vi "Test_case.vi"(7 "base path":path=path "D:/1.INPROGRESS/16.Ather/6.Software/Ather_ANC_LEV_Labview_Software/Template", 9 "Main Test Status":refnum<vi>, 10 "queue out":refnum<queue>, 11 "Data Cluster":T2={"Boolean <Replace Me>"=FALSE, "String <Replace Me>"="", "Numeric <Replace Me>"=0.0, "Do Something Ref"=refnum, "Do Something Else Ref"=refnum, "Data Display Ref"=refnum, "Exit Button Ref"=refnum, "Enum"=enum."Admin", "skip Test  "=[]}) -> (3 "Result":string[][](array[string]))   [LabVIEW 2021]
uses:
  controls/UI Data.ctl
  Main_VI/Control/login_type.ctl
  controls/Main test sequence.ctl
  5.ACTIVITIES/1.LabVIEW_State_Machine_Template/LabVIEW_State_Machine_Template/LabVIEW_State_Machine_Template/Project_Template/Queue Test updator/Controls/initialise cluster.ctl
  5.ACTIVITIES/1.LabVIEW_State_Machine_Template/LabVIEW_State_Machine_Template/LabVIEW_State_Machine_Template/Project_Template/Queue Test updator/Controls/test step description.ctl
  5.ACTIVITIES/1.LabVIEW_State_Machine_Template/LabVIEW_State_Machine_Template/LabVIEW_State_Machine_Template/Project_Template/Queue Test updator/Controls/comparison selection.ctl
panel:
  out "Main test sequence 2":T1
  out "Main test sequence":T1
  out "s? t:f":T1
  out "Test Status 2":i32(listbox)=-1
  out "UI":string[][](array[string])=[["1", "start BB4 card auto testing", "0.000", "0.000", "", ""], ["2", "scan barcode", "0.000", "0.000", "", ""], ["3", "ensure resistor settings", "0.000", "0.000", "", ""], ["4", "check shorting of TP01 wrt GND", "100000.000", "200000.000", "", ""], ["5", "check shorting of TP02 wrt GND", "100000.000", "200000.000", "", ""], ["6", "check shorting of TP05 wrt GND", "100000.000", "200000.000", "", ""], ["7", "check shorting of TP36 wrt GND", "180.000", "200.000", "", ""], ["8", "check shorting of TP42 wrt GND", "240.000", "270.000", "", ""], ["9", "check shorting of TP41 wrt GND", "210.000", "230.000", "", ""], ["10", "check shorting of TP30 wrt GND", "145.000", "155.000", "", ""], ["11", "turn ON 5V PS", "0.000", "0.000", "", ""], ["12", "measure voltage at TP01", "3.200", "3.400", "", ""], ["13", "measure voltage at TP02", "3.200", "3.400", "", ""], ["14", "measure voltage at TP05", "1.600", "1.800", "", ""], ["15", "measure 0.02A current at PS_I/P", "0.010", "0.030", "", ""], ["16", "program UCD9081(JF1)", "0.100", "0.300", "", ""], ["17", "program UCD9081(JF2)", "0.000", "0.000", "", ""], ["18", "program UCD9081(JF3)", "0.000", "0.000", "", ""], ["19", "measure 0.4A current at PS_I/P", "0.350", "0.450", "", ""], ["20", "turn OFF 5V PS", "0.000", "0.000", "", ""], ["21", "measure resistance at C56_C59", "100000.000", "200000.000", "", ""], ["22", "turn ON 5V PS", "0.000", "0.000", "", ""], ["23", "measure voltage at TP36", "1.700", "1.900", "", ""], ["24", "measure voltage at TP42", "3.200", "3.400", "", ""], ["25", "measure voltage at TP41", "1.100", "1.300", "", ""], ["26", "measure voltage at TP30", "2.400", "2.600", "", ""], ["27", "boundary scan test", "0.000", "0.000", "", ""], ["28", "monitor clock I/P of U49.3", "26.500", "27.500", "", ""], ["29", "flash Cypress_CY223811FXI", "0.000", "0.000", "", ""], ["30", "monitor clock I/P of U48.1", "24.500", "25.500", "", ""], ["31", "monitor clock I/P of U48.5", "26.500", "27.500", "", ""], ["32", "monitor clock I/P of U32.2", "24.500", "25.500", "", ""], ["33", "monitor clock I/P of U32.3", "24.500", "25.500", "", ""], ["34", "monitor clock I/P of U32.4", "24.500", "25.500", "", ""], ["35", "monitor clock I/P of U32.5", "24.500", "25.500", "", ""], ["36", "monitor clock I/P of U53.2", "24.500", "25.500", "", ""], ["37", "monitor clock I/P of U53.3", "24.500", "25.500", "", ""], ["38", "monitor clock I/P of U53.4", "24.500", "25.500", "", ""], ["39", "monitor clock I/P of U53.5", "24.500", "25.500", "", ""], ["40", "monitor clock I/P of U233.2", "24.500", "25.500", "", ""], ["41", "monitor clock I/P of U233.3", "24.500", "25.500", "", ""], ["42", "monitor clock I/P of U233.4", "24.500", "25.400", "", ""], ["43", "monitor clock I/P of U233.5", "24.500", "25.500", "", ""], ["44", "monitor clock I/P of U33.2", "26.500", "27.500", "", ""], ["45", "monitor clock I/P of U33.3", "26.500", "27.500", "", ""], ["46", "monitor clock I/P of U33.4", "26.500", "27.500", "", ""], ["47", "monitor clock I/P of U33.5", "26.500", "27.500", "", ""], ["48", "monitor clock I/P of U38.2", "26.500", "27.500", "", ""], ["49", "monitor clock I/P of U38.3", "26.500", "27.500", "", ""], ["50", "monitor clock I/P of U38.4", "26.500", "27.500", "", ""], ["51", "monitor clock I/P of U38.5", "26.500", "27.500", "", ""], ["52", "monitor clock I/P of U46.2", "26.500", "27.500", "", ""], ["53", "monitor clock I/P of U46.3", "26.500", "27.500", "", ""], ["54", "monitor clock I/P of U46.4", "26.500", "27.500", "", ""], ["55", "monitor clock I/P of U46.5", "26.500", "27.500", "", ""], ["56", "monitor reset O/P of U60.1 as 5.0V", "4.800", "5.200", "", ""], ["57", "monitor reset O/P of U36.4 as 5.0V", "4.800", "5.200", "", ""], ["58", "monitor reset O/P of U36.6 as 5.0V", "4.800", "5.200", "", ""], ["59", "monitor reset O/P of U36.8 as 5.0V", "4.800", "5.200", "", ""], ["60", "monitor reset O/P of U36.10 as 5.0V", "4.800", "5.200", "", ""], ["61", "monitor reset O/P of U36.12 as 5.0V", "4.800", "5.200", "", ""], ["62", "user prompt for pressing reset switch SW3 at U60.1", "0.000", "0.000", "", ""], ["63", "user prompt for pressing reset switch SW3 at U36.4", "0.000", "0.000", "", ""], ["64", "user prompt for pressing reset switch SW3 at U36.6", "0.000", "0.000", "", ""], ["65", "user prompt for pressing reset switch SW3 at U36.8", "0.000", "0.000", "", ""], ["66", "user prompt for pressing reset switch SW3 at U36.10", "0.000", "0.000", "", ""], ["67", "user prompt for pressing reset switch SW3 at U36.12", "0.000", "0.000", "", ""], ["68", "program FPGA via .bit file", "0.000", "0.000", "", ""], ["69", "FPGA SPI flash via .mcs file", "0.000", "0.000", "", ""], ["70", "Ethernet test_Portxx", "0.000", "0.000", "", ""], ["71", "JTAG connectivity of DAVINCI (SMS320DM6446AZWTA)", "0.000", "0.000", "", ""], ["72", "UBOOT test_DVflasher", "0.000", "0.000", "", ""], ["73", "UBOOT test_send command on hyperterminal and verify result", "0.000", "0.000", "", ""], ["74", "Send Kernel_INDESDR", "0.000", "0.000", "", ""], ["75", "Send NAND Erase_Write_Boot", "0.000", "0.000", "", ""], ["76", "Send_nci_nce_ncn", "0.000", "0.000", "", ""], ["77", "Muti IDE", "0.000", "0.000", "", ""], ["78", "FileZilla File System Transfer", "0.000", "0.000", "", ""], ["79", "Telnet Unmount Device", "0.000", "0.000", "", ""], ["80", "Ethernet test_Portxx", "0.000", "0.000", "", ""], ["81", "LAN9250 test", "0.000", "0.000", "", ""], ["82", "ping IP_LAN9250 test", "0.000", "0.000", "", ""], ["83", "RTC Test", "0.000", "0.000", "", ""], ["84", "Shared Memory Test", "0.000", "0.000", "", ""], ["85", "Temperature_Sensor_Test", "0.000", "0.000", "", ""], ["86", "GPS_Test", "0.000", "0.000", "", ""], ["87", "External Clock Test", "0.000", "0.000", "", ""], ["88", "stop BB4 card auto testing", "0.000", "0.000", "", ""]]
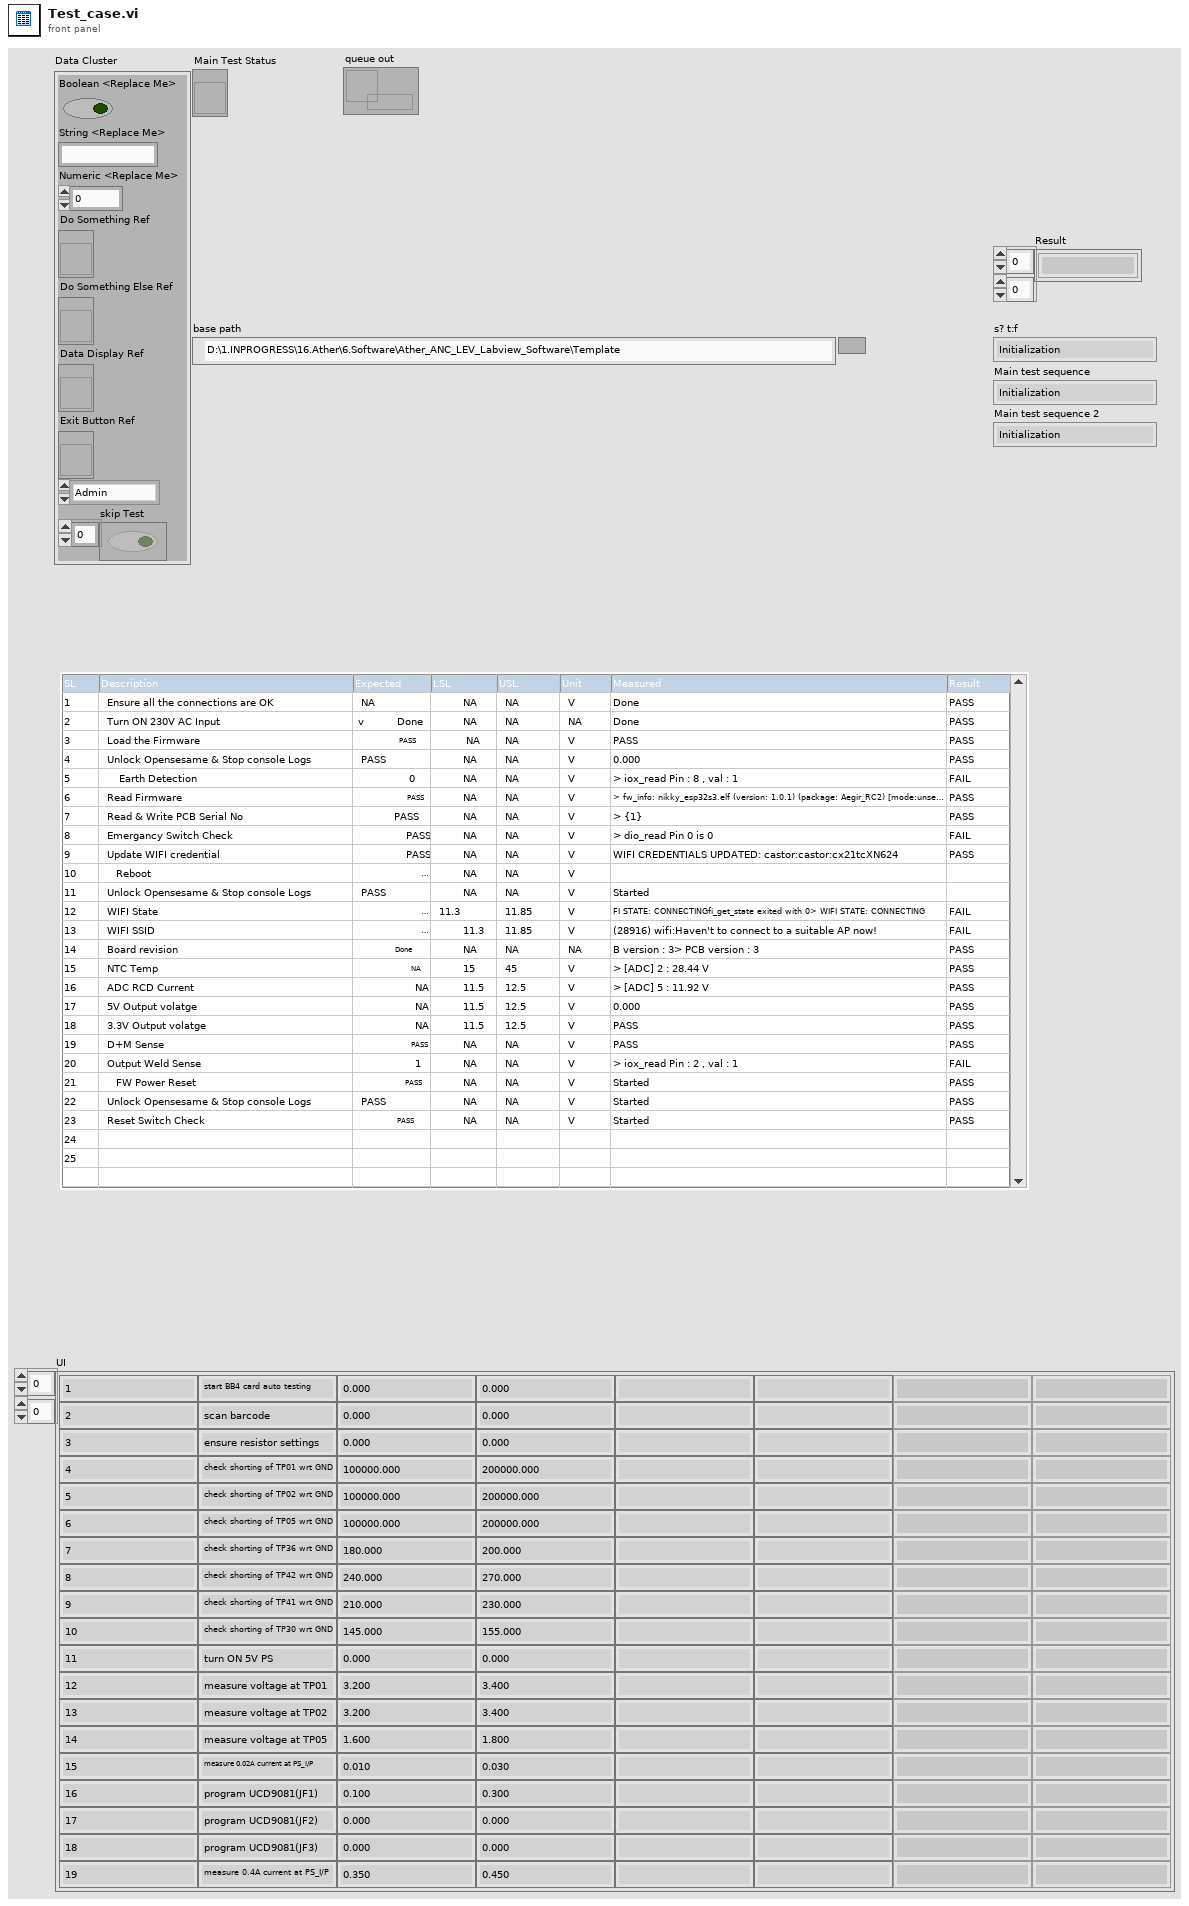
[diagram p1: front panel]
types:
  T1 = typedef "Main test sequence.ctl" = enum16{"Initialization", "Ensure all the connections are OK", "Turn ON 230V AC Input", "Load the Firmware", "Unlock_Opensesame & Stop console Logs", "Earth Detection", "Read Firmware", "Read & Write PCB Serial No", "Emergancy Switch Check", "Update WIFI credentials ", "Reboot", "Unlock Opensesame & Stop_console Logs", "WIFI State", "WIFI SSID", "Board revision", "ADC NTC Temp", "ADC_TYPE2_RCD_CURRENT", "5V Output Voltage", "3.3V Output Voltage", "D+M Sense", "Output Weld Sense", "FW Power Reset", "Unlock Opensesame & Stop console_Logs", "Reset switch Check", "Exit"}
  T2 = typedef "UI Data.ctl" = cluster{"Boolean <Replace Me>":bool, "String <Replace Me>":string, "Numeric <Replace Me>":dbl, "Do Something Ref":refnum<vi>, "Do Something Else Ref":refnum<vi>, "Data Display Ref":refnum<vi>, "Exit Button Ref":refnum<vi>, "Enum":T3, "skip Test  ":bool[]}
  T3 = typedef "login_type.ctl" = enum16{"Operator", "Admin"}
  T4 = typedef "initialise cluster.ctl" = cluster{"User name":string, "user account":string, "UI":string[][], "DI":T5[], "Barcode":string, "MCListbox Ref_in":refnum<vi>, "sequence step #":u32, "Result?":bool, "Report Path":path, "Test Sequence":T1, "skip Test  ":bool[]}
  T5 = typedef "test step description.ctl" = cluster{"Lower limit":dbl, "Upper limit":dbl, "Comparison":T6, "Expected":string, "Enable":bool, "Main test sequence":T1}
  T6 = typedef "comparison selection.ctl" = enum16{"None", "in-range?", "less than?", "greater than?", "equal to?", "not equal to?", "less or equal to?", "greater or equal to?"}
  T7 = typedef "initialise cluster.ctl" = cluster{"User name":string, "user account":string, "UI":string[][], "DI":T8[], "Skip test?":bool[], "Barcode":string, "MCListbox Ref_in":refnum<vi>, "sequence step #":u32, "Result?":bool, "Report Path":path, "Enum":T10}
  T8 = typedef "test step description.ctl" = cluster{"Test_Sequence":T9, "Lower limit":dbl, "Upper limit":dbl, "Comparison":T6, "Expected":string, "Enable":bool}
  T9 = typedef "Test_sequence.ctl" = enum16{"Init Devices", "Login", "Option Window", "Idle state", "Scan Barcode", "Clear the test Containers", "Init-Pre Test", "Test ", "Result", "Report", "Database", "Update Display", "Confirm Quit", "Error", "Exit"}
  T10 = typedef "Test_Sequence_4.ctl" = enum16{"Update Display", "User Login", "Operator", "Admin", "Developer", "Update Test Seq", "Initialise", "Init Devices", "Idle State", "Check All", "UnCheck All", "Abort", "Start Testing", "Turn ON Power", "Scan Barcode", "POP to place DUT", "Toggle Operation confirmation", "Error", "Confirm Quit", "Exit", "Code flash", "Operating Voltage range test", "Under Voltage Protection", "Reverse Voltage Test at 28V", "Reverse Voltage Recovery", "Output Test at 8V", "Output Test at 9V", "Output Test at 10V", "Output Test at 11V", "Output Test at 12V", "Output Test at 15V", "Output Test at 24V", "Output Test at 32V", "Video Signal Conversion Test", "USB Interface Verification", "Turn OFF Power", "Report"}
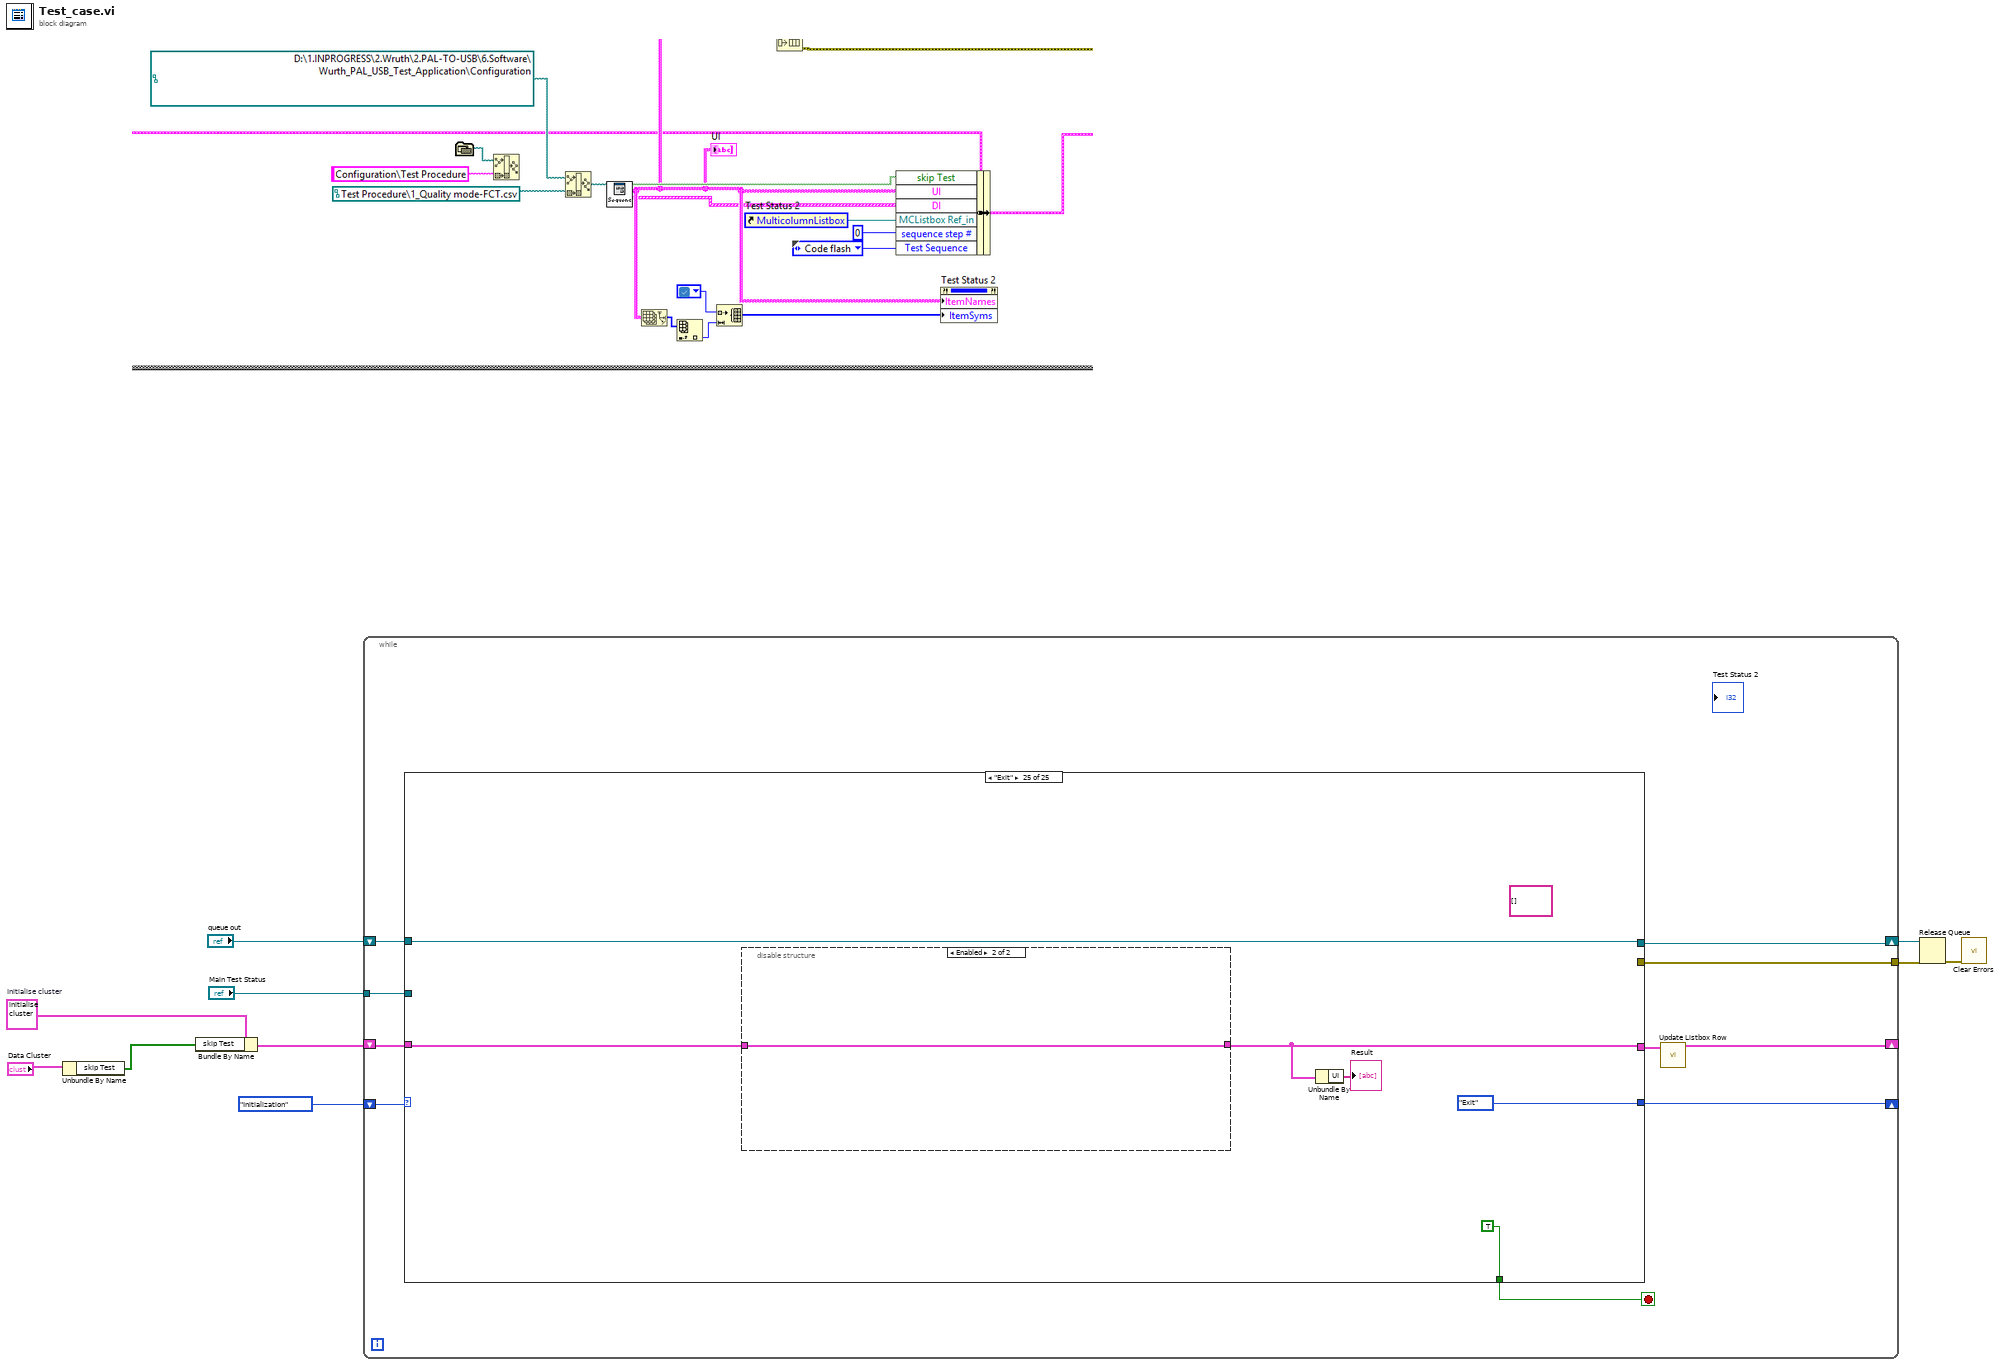
[diagram p0: block diagram]
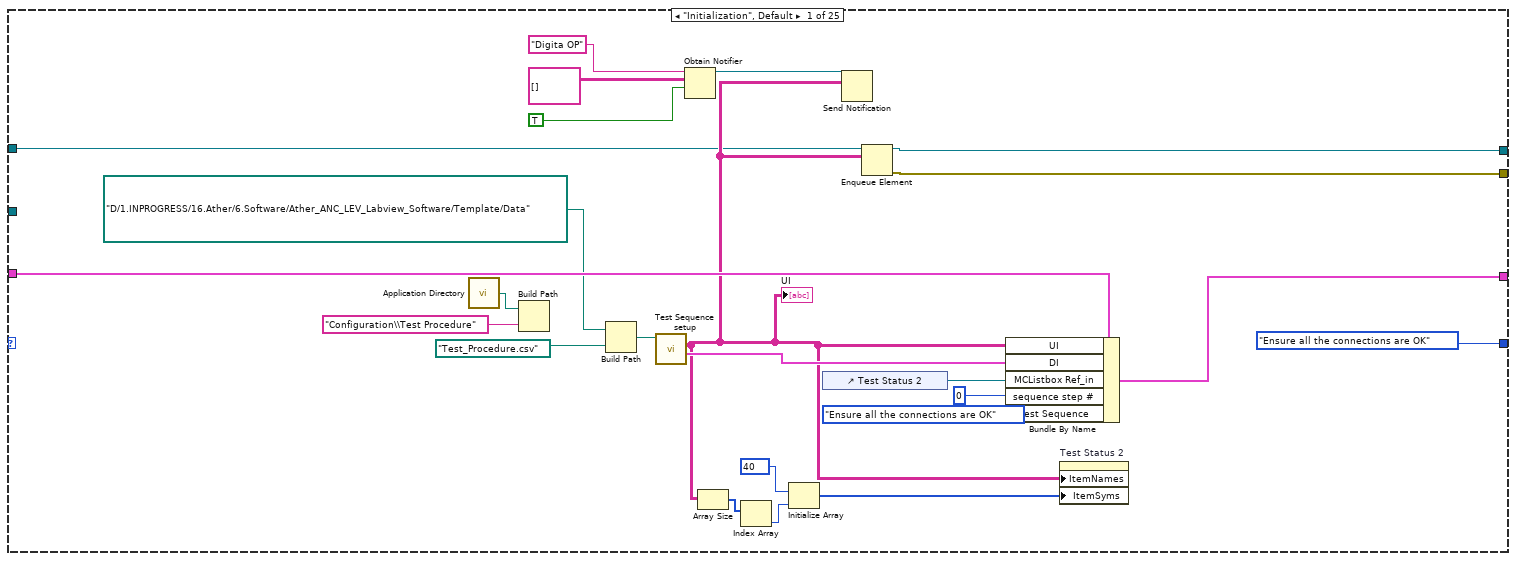
[diagram p2: hidden frame]
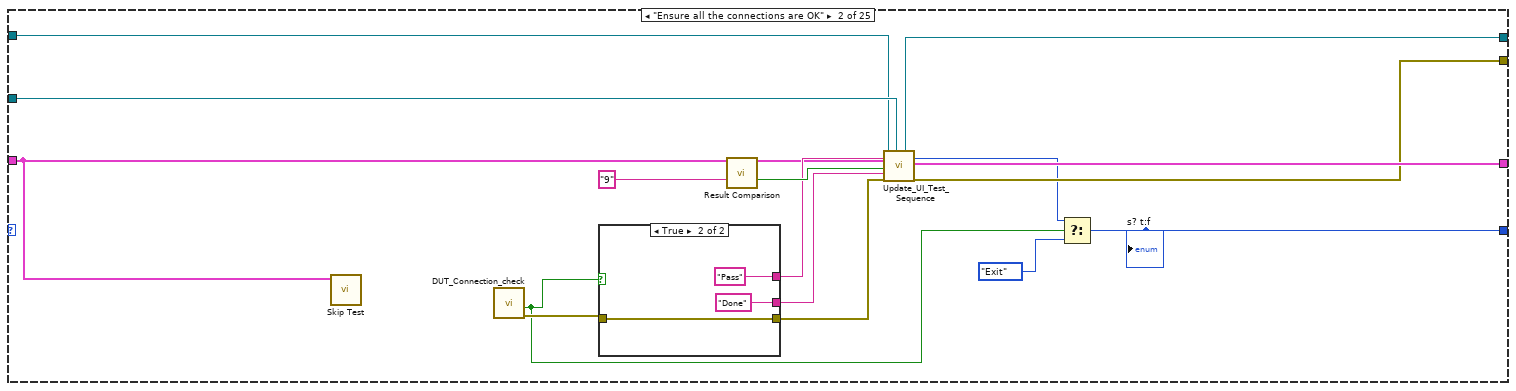
[diagram p3: hidden frame]
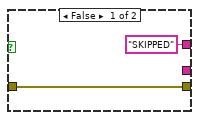
[diagram p4: hidden frame]
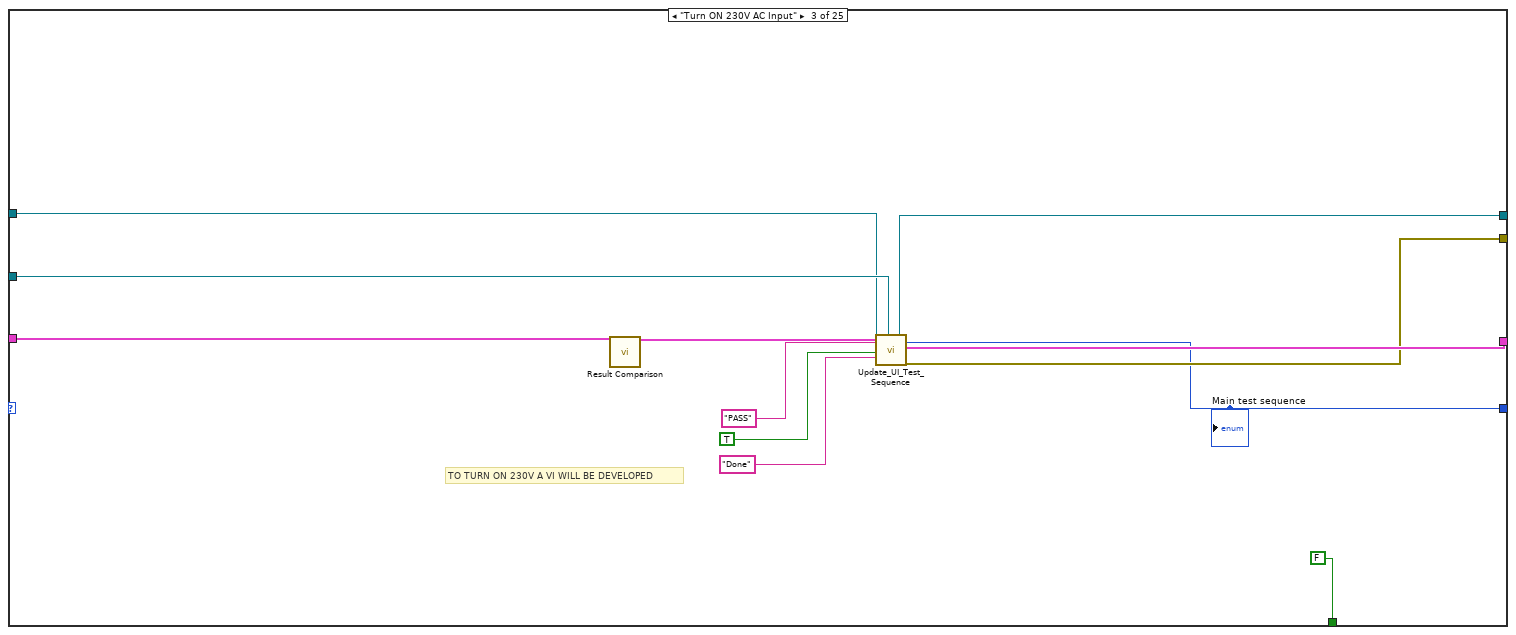
[diagram p5: hidden frame]
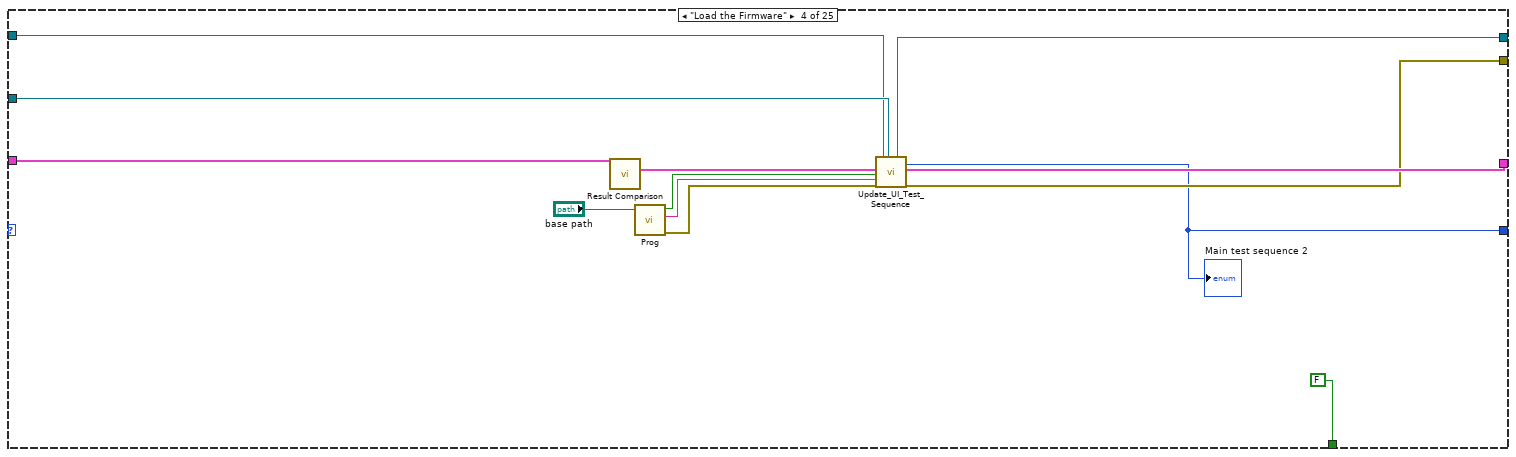
[diagram p6: hidden frame]
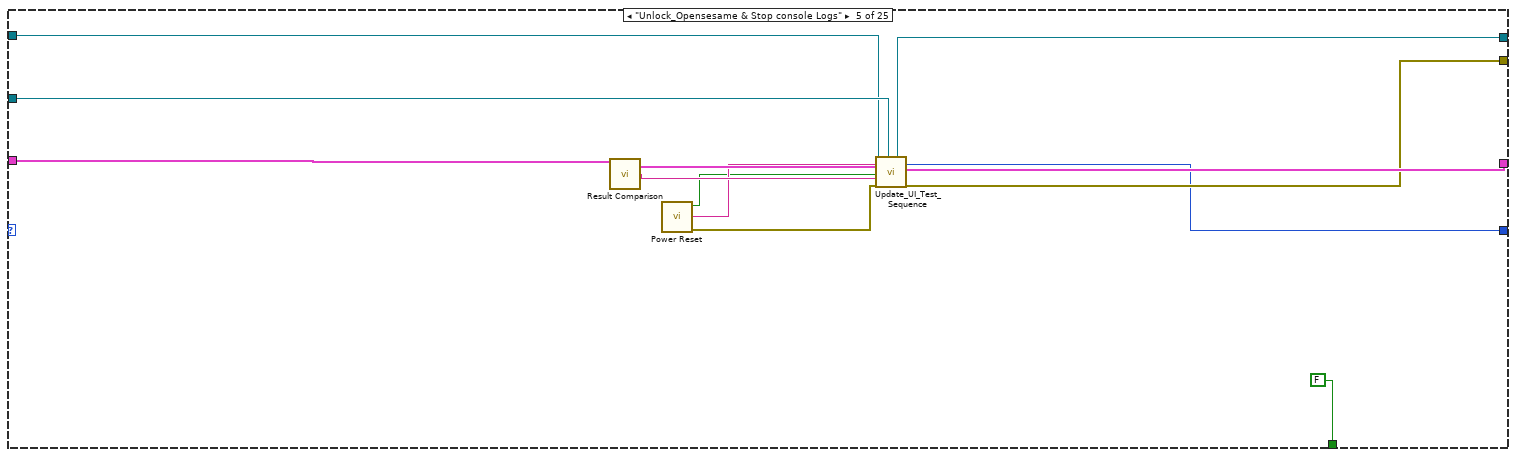
[diagram p7: hidden frame]
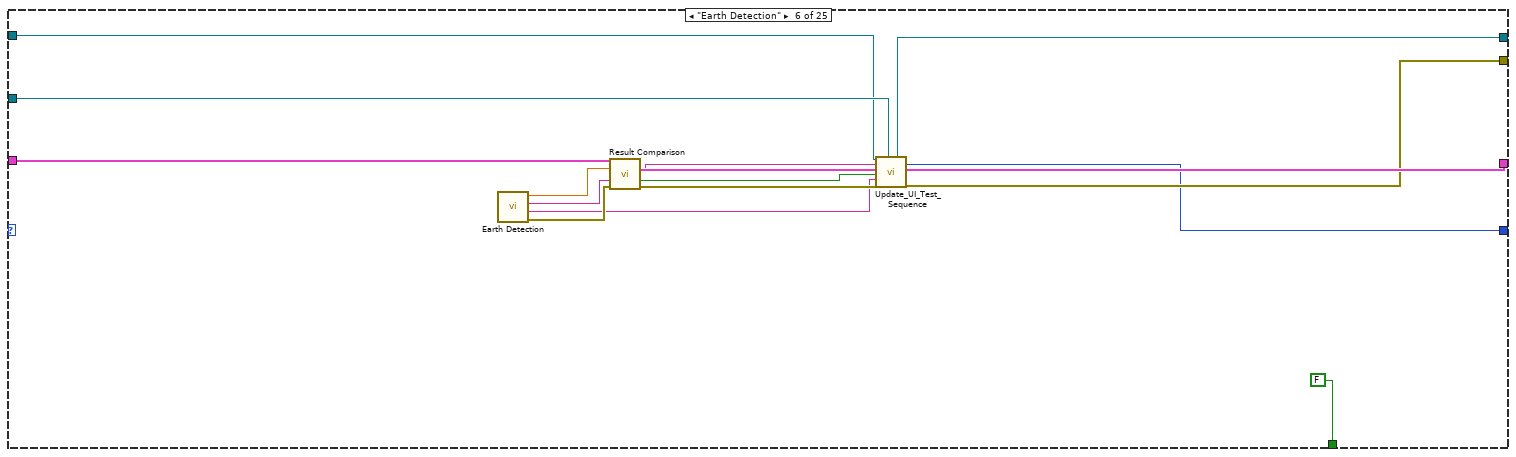
[diagram p8: hidden frame]
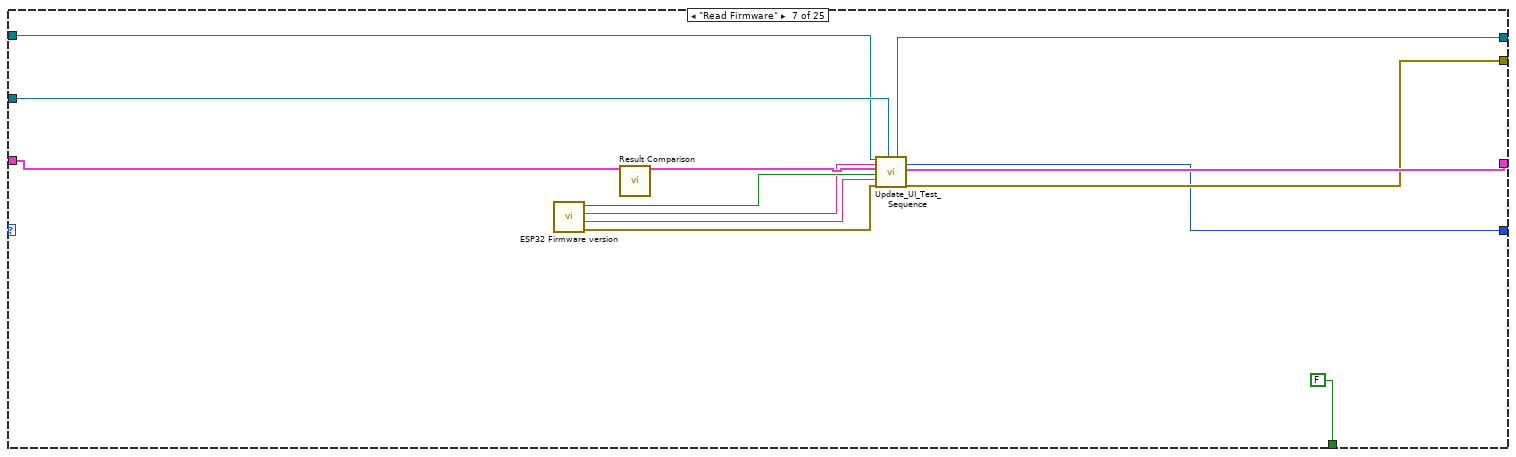
[diagram p9: hidden frame]
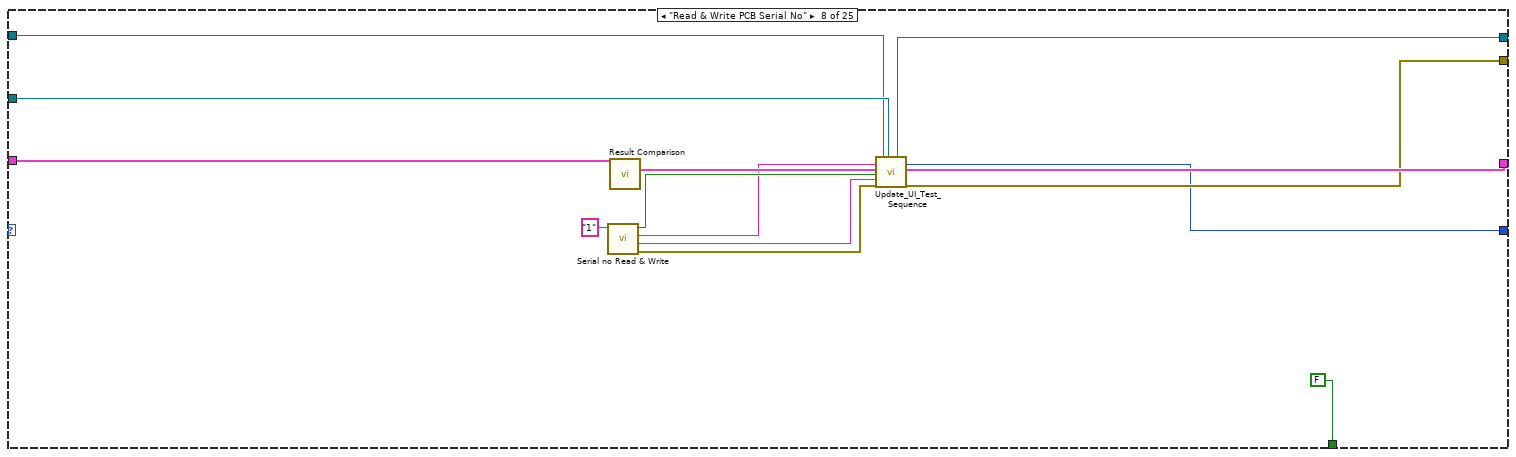
[diagram p10: hidden frame]
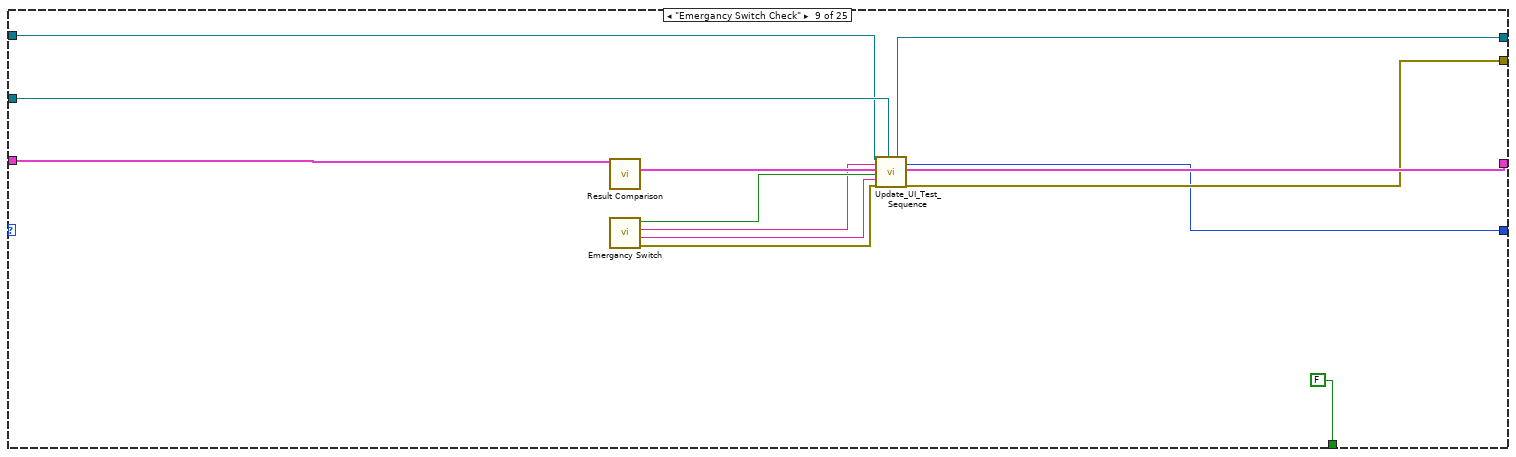
[diagram p11: hidden frame]
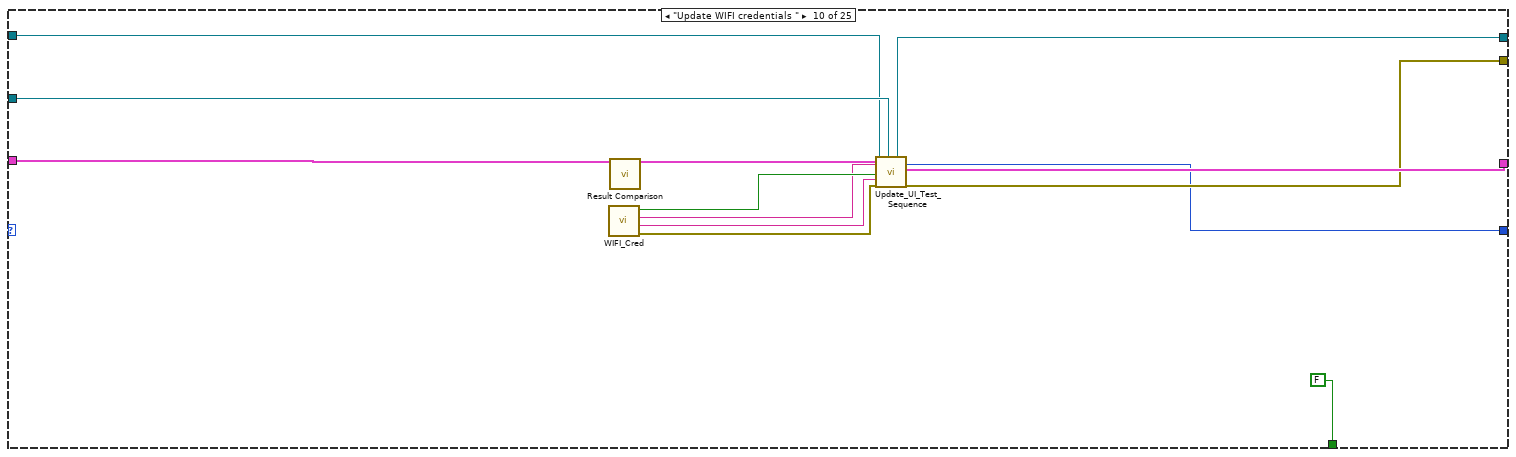
[diagram p12: hidden frame]
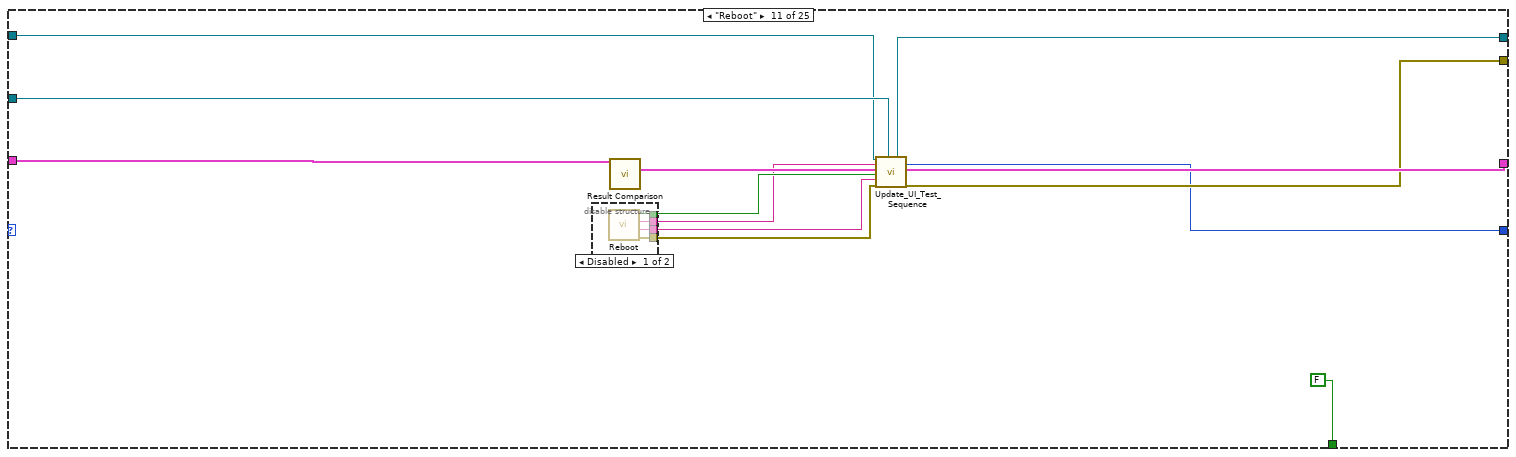
[diagram p13: hidden frame]
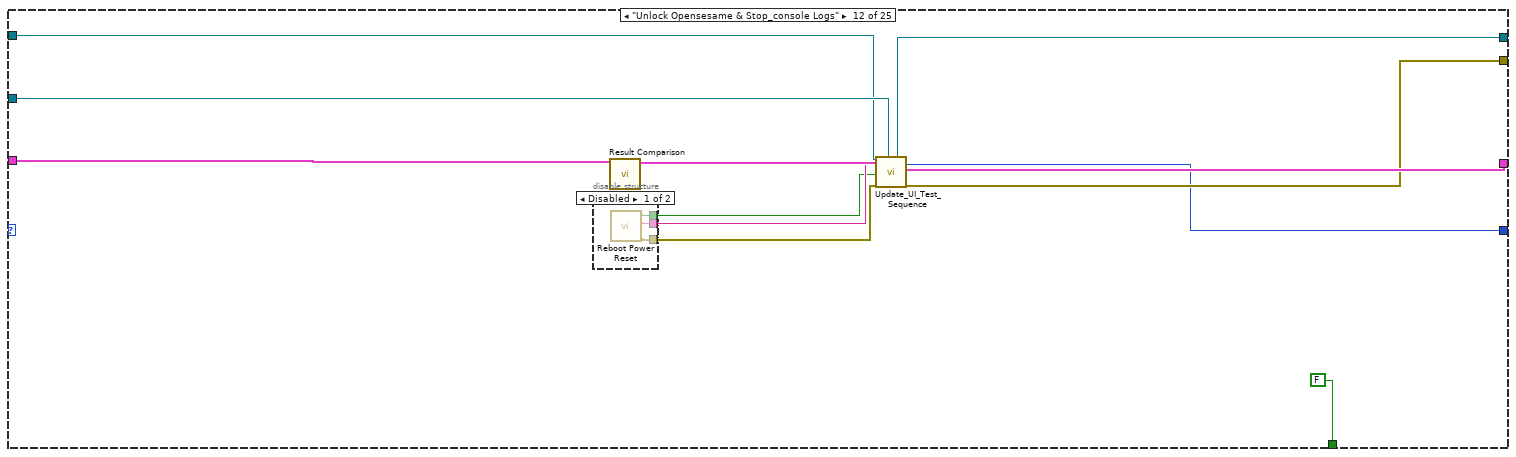
[diagram p15: hidden frame]
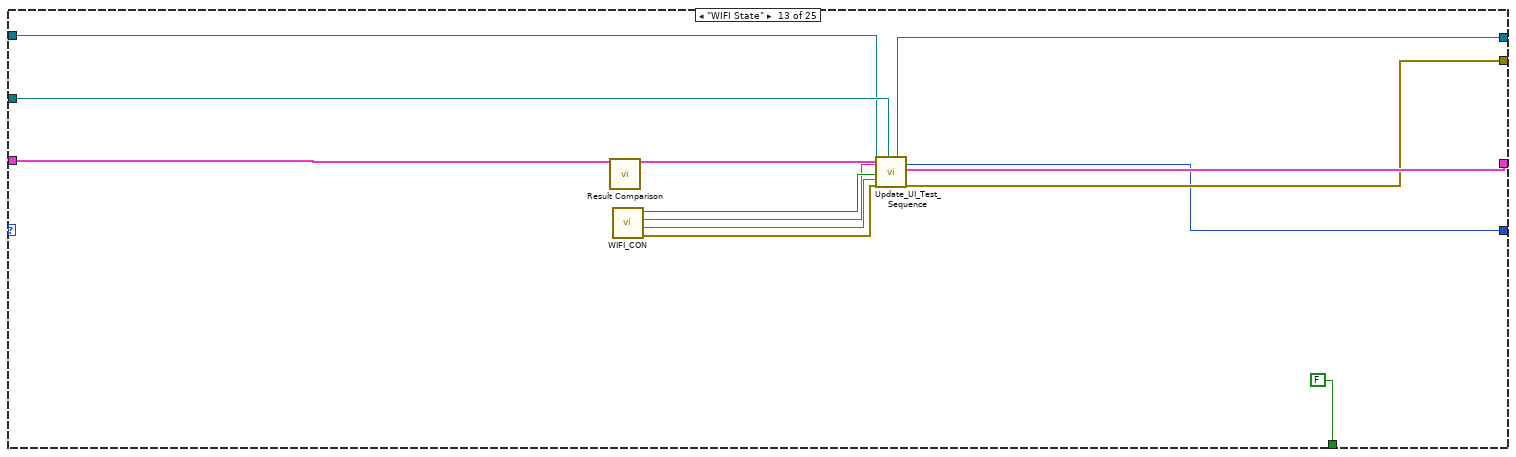
[diagram p17: hidden frame]
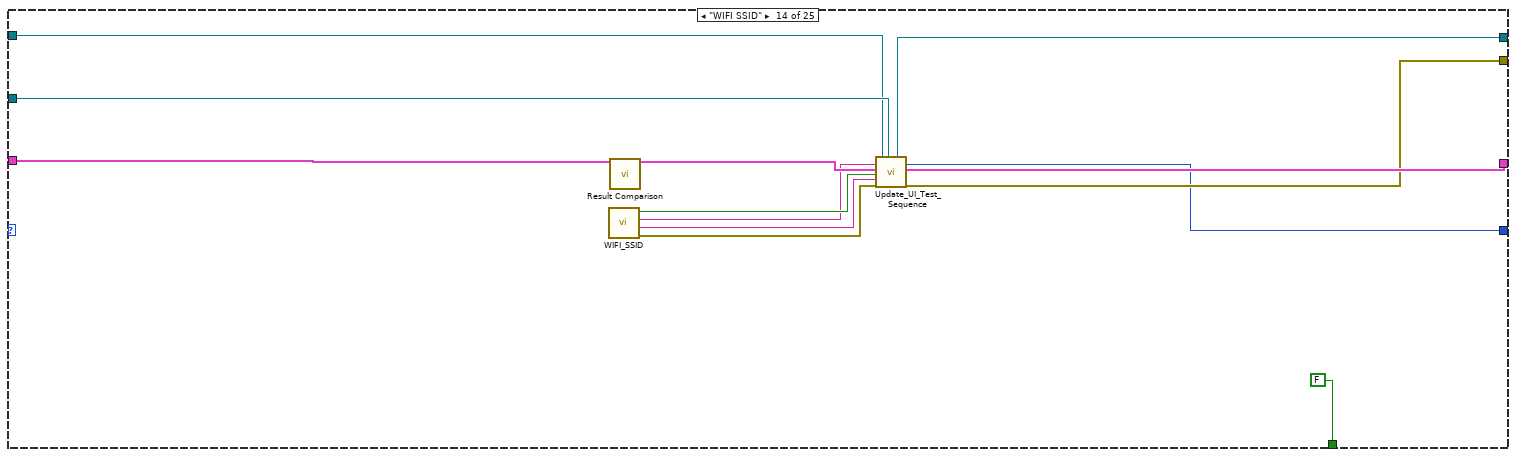
[diagram p18: hidden frame]
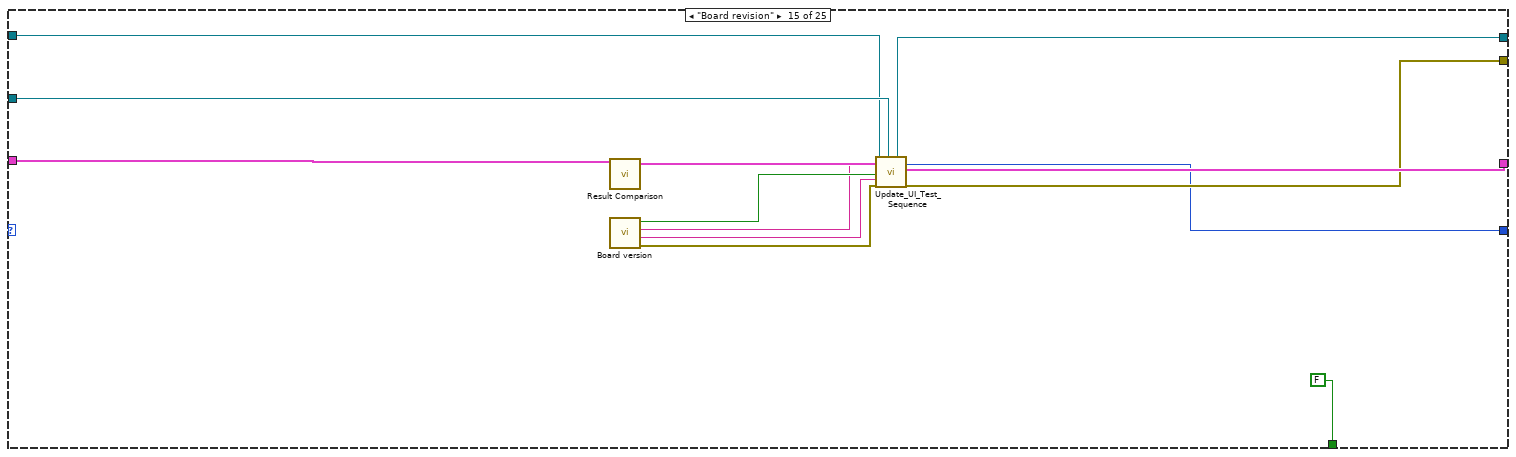
[diagram p19: hidden frame]
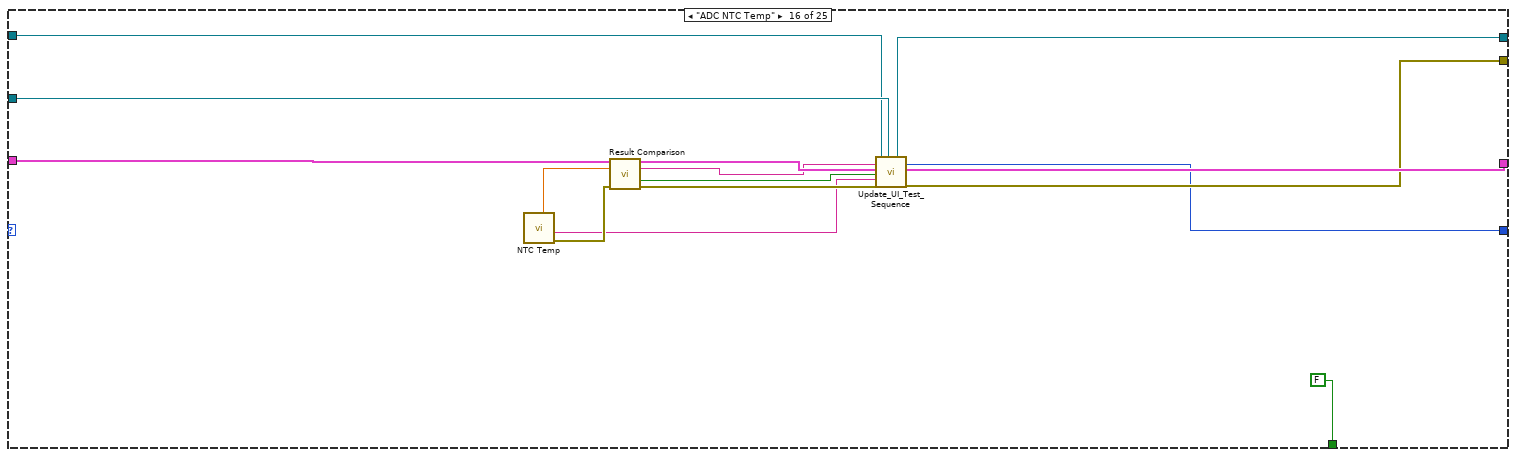
[diagram p20: hidden frame]
diagram:
  w6 = T4 {"User name"="", "user account"="", "UI"=[], "DI"=[], "Barcode"="", "MCListbox Ref_in"=refnum, "sequence step #"=0, "Result?"=FALSE, "Report Path"=path "", "Test Sequence"=enum."Ensure all the connections are OK", "skip Test  "=[FALSE, FALSE, FALSE, FALSE, FALSE, FALSE, FALSE, FALSE, FALSE, FALSE, FALSE, FALSE, FALSE, FALSE, FALSE, FALSE, FALSE, FALSE, FALSE, FALSE, FALSE, FALSE, FALSE, FALSE, FALSE, FALSE, FALSE, FALSE, FALSE, FALSE, FALSE, FALSE]}  # Initialise cluster
  n1 = Unbundle By Name("Data Cluster") -> ("skip Test"=w5:bool[])
  n2 = Bundle By Name(cluster=w6, "skip Test"=w5) -> (w4:T4)
  n3 = while {
    shift-right: [w20] -> _
    shift-left: w4 -> [w18]
    shift-right: [w16] -> w8
    shift-left: "queue out" -> [w11]
    tunnel: "Main Test Status" -> [w15]
    tunnel: [w14] -> w7
    shift-right: [w12] -> _
    shift-left: Main_test_sequence."Initialization" -> [w13]
    stop <- w17 stop-if-true
    n4 = case shown="\"Exit\"" w13 {
      tunnel: w18 -> [w39 w54 w78 w91 w104 w120 w133 w147 w160 w173 w186 w202 w218 w231 w244 w259 w273 w285 w296 w307 w323 w334 w346 w361 w367]
      tunnel: [w24 w57 w77 w90 w103 w119 w132 w146 w159 w172 w185 w201 w217 w230 w243 w258 w272 w284 w295 w306 w322 w333 w345 w360 w364] -> w19
      tunnel: [Main_test_sequence."Ensure all the connections are OK" w46 w71 w86 w98 w115 w128 w142 w155 w168 w181 w197 w213 w226 w239 w254 w268 w278 w291 w302 w318 w328 w341 w356 Main_test_sequence."Exit"] -> w12
      tunnel: [_ _ FALSE FALSE FALSE FALSE FALSE FALSE FALSE FALSE FALSE FALSE FALSE FALSE FALSE FALSE FALSE FALSE FALSE FALSE FALSE FALSE FALSE FALSE TRUE] -> w17
      tunnel: [w31 w56 w73 w88 w100 w117 w130 w144 w157 w170 w183 w199 w215 w228 w241 w256 w270 w281 w293 w304 w320 w331 w343 w358 w362] -> w16
      tunnel: [w30 w55 w72 w87 w99 w116 w129 w143 w156 w169 w182 w198 w214 w227 w240 w255 w269 w280 w292 w303 w319 w330 w342 w357 _] -> w14
      tunnel: w15 -> [_ w53 w70 w85 w97 w114 w127 w141 w154 w167 w180 w196 w212 w225 w238 w253 w267 w277 w290 w301 w317 w327 w340 w355 _]
      tunnel: w11 -> [w21 w45 w67 w79 w92 w105 w121 w134 w148 w161 w174 w191 w206 w219 w232 w245 w260 w274 w286 w297 w309 w324 w335 w350 w362]
      frame "Initialization", Default {
        n5 = call <vilib>:"Application Directory.vi"() -> ("Application Directory"=w43:path)
        n6 = Build Path(base path=w43, name or relative path="Configuration\\Test Procedure") -> ()  [unwired: 1 out]
        n7 = Build Path(base path=path "D:/1.INPROGRESS/16.Ather/6.Software/Ather_ANC_LEV_Labview_Software/Template/Data", name or relative path=path "Test_Procedure.csv") -> (appended path=w41:path)
        n8 = call "Test Sequence setup.vi"("Test Procedure Path"=w41) -> ("DI 2"=w36:T5[], "UI"=w26:string[][])  [unwired: 7 in, 2 out]
        "UI" <- w26
        n9 = Obtain Notifier(name (unnamed)="Digita OP", notification data type=string[][] [] ("Test status item names"), create if not found? (T)=TRUE) -> (notifier out=w35:refnum<notifier>)  [unwired: 1 in, 2 out]
        n10 = Array Size(array=w26) -> (size(s)=w29:i32[])
        n11 = Index Array(array=w29) -> (element=w28:i32)  [unwired: 1 in]
        n12 = Initialize Array(40, w28) -> (w25:i32[])
        n13 = control-ref of="Test Status 2"() -> (w44:refnum<vi>)
        n14 = Send Notification(notification=w26, notifier=w35) -> ()  [unwired: 1 in, 2 out]
        n15 = Enqueue Element(queue=w21, element=w26) -> (queue out=w31:refnum<queue>, error out=w30:errorcluster)  [unwired: 2 in, 1 out]
        n16 = Bundle By Name(cluster=w39, "UI"=w26, "DI"=w36, "MCListbox Ref_in"=w44, "sequence step #"=u32 0, "Test Sequence"=Main_test_sequence."Ensure all the connections are OK") -> (w24:T4)
        n17 = property on="Test Status 2" class="MCListbox (strict)"("ItemNames"=w26, "ItemSyms"=w25) -> ()  [unwired: 2 in, 2 out]
      }
      frame "Ensure all the connections are OK" {
        n18 = call "Skip Test.vi"("Initialise cluster"=w54) -> ()  [unwired: 10 in, 1 out]
        n19 = call "DUT_Connection_check.vi"() -> ("error out"=w51:errorcluster, "PASS"=w48:bool)  [unwired: 10 in]
        n20 = case shown="True" w48 {
          tunnel: [_ "Done" ("measured value")] -> w59
          tunnel: ["SKIPPED" ("result") "Pass" ("result")] -> w58
          tunnel: w51 -> [w63 w64]
          tunnel: [w63 w64] -> w50
          frame False {
          }
          frame True {
          }
        }
        n21 = call "Result Comparison.vi"("input cluster"=w54, "Measued String"="9") -> ("Output cluster"=w52:T4, "result?"=w61:bool)  [unwired: 9 in, 3 out]
        n22 = call "Update_UI_Test_Sequence.vi"("queue out 2"=w45, "result"=w58, "input cluster"=w52, "Result"=w61, "measured value"=w59, "error in"=w50, "Main Test Status"=w53) -> ("queue out"=w56:refnum<queue>, "Main test sequence"=w49:T1, "output cluster"=w57:T4, "error out"=w55:errorcluster)  [unwired: 9 in]
        n23 = Select(t=w49, s=w48, f=Main_test_sequence."Exit") -> (s? t:f=w46:T1)
        "s? t:f" <- w46
      }
      frame "Turn ON 230V AC Input" {
        # "TO TURN ON 230V A VI WILL BE DEVELOPED"
        n24 = call "Result Comparison.vi"("input cluster"=w78) -> ("Output cluster"=w69:T4)  [unwired: 10 in, 4 out]
        n25 = call "Update_UI_Test_Sequence.vi"("queue out 2"=w67, "result"="PASS", "input cluster"=w69, "Result"=TRUE, "measured value"="Done", "Main Test Status"=w70) -> ("queue out"=w73:refnum<queue>, "Main test sequence"=w71:T1, "output cluster"=w77:T4, "error out"=w72:errorcluster)  [unwired: 10 in]
        "Main test sequence" <- w71
      }
      frame "Load the Firmware" {
        n26 = call "Result Comparison.vi"("input cluster"=w91) -> ("Output cluster"=w84:T4)  [unwired: 10 in, 4 out]
        n27 = call "Prog.vi"("base path"="base path") -> ("error out"=w81:errorcluster, "Result"=w83:string, "RESULT"=w82:bool)  [unwired: 6 in]
        n28 = call "Update_UI_Test_Sequence.vi"("queue out 2"=w79, "input cluster"=w84, "Result"=w82, "measured value"=w83, "error in"=w81, "Main Test Status"=w85) -> ("queue out"=w88:refnum<queue>, "Main test sequence"=w86:T1, "output cluster"=w90:T4, "error out"=w87:errorcluster)  [unwired: 10 in]
        "Main test sequence 2" <- w86
      }
      frame "Unlock_Opensesame & Stop console Logs" {
        n29 = call "Result Comparison.vi"("input cluster"=w104) -> ("Output cluster"=w96:T4, "measured value"=w101:string)  [unwired: 10 in, 3 out]
        n30 = call "Power Reset.vi"() -> ("error out"=w95:errorcluster, 2:"Result"=w94:string, 3:"Result"=w93:bool)  [unwired: 9 in]
        n31 = call "Update_UI_Test_Sequence.vi"("queue out 2"=w92, "result"=w94, "input cluster"=w96, "Result"=w93, "measured value"=w101, "error in"=w95, "Main Test Status"=w97) -> ("queue out"=w100:refnum<queue>, "Main test sequence"=w98:T1, "output cluster"=w103:T4, "error out"=w99:errorcluster)  [unwired: 9 in]
      }
      frame "Earth Detection" {
        n32 = call "Earth Detection.vi"() -> ("error out"=w107:errorcluster, "Command Response"=w106:string, "Measured Data"=w108:string, "number"=w109:dbl)  [unwired: 6 in]
        n33 = call "Result Comparison.vi"("input cluster"=w120, "measured data"=w109, "Measued String"=w108, "error in (no error)"=w107) -> ("Output cluster"=w113:T4, "result"=w110:string, "result?"=w112:bool, "error out"=w111:errorcluster)  [unwired: 7 in, 1 out]
        n34 = call "Update_UI_Test_Sequence.vi"("queue out 2"=w105, "result"=w110, "input cluster"=w113, "Result"=w112, "measured value"=w106, "error in"=w111, "Main Test Status"=w114) -> ("queue out"=w117:refnum<queue>, "Main test sequence"=w115:T1, "output cluster"=w119:T4, "error out"=w116:errorcluster)  [unwired: 9 in]
      }
      frame "Read Firmware" {
        n35 = call "ESP32 Firmware version.vi"() -> ("error out"=w125:errorcluster, "Command Response"=w122:string, "Result"=w123:string, "RESULT"=w124:bool)  [unwired: 8 in]
        n36 = call "Result Comparison.vi"("input cluster"=w133) -> ("Output cluster"=w126:T4)  [unwired: 10 in, 4 out]
        n37 = call "Update_UI_Test_Sequence.vi"("queue out 2"=w121, "result"=w123, "input cluster"=w126, "Result"=w124, "measured value"=w122, "error in"=w125, "Main Test Status"=w127) -> ("queue out"=w130:refnum<queue>, "Main test sequence"=w128:T1, "output cluster"=w132:T4, "error out"=w129:errorcluster)  [unwired: 9 in]
      }
      frame "Read & Write PCB Serial No" {
        n38 = call "Serial no Read & Write.vi"("PCB Serial No"="1") -> ("error out"=w139:errorcluster, "Command Response"=w137:string, "Result"=w135:string, "RESULT"=w136:bool)  [unwired: 7 in]
        n39 = call "Result Comparison.vi"("input cluster"=w147) -> ("Output cluster"=w140:T4)  [unwired: 10 in, 4 out]
        n40 = call "Update_UI_Test_Sequence.vi"("queue out 2"=w134, "result"=w135, "input cluster"=w140, "Result"=w136, "measured value"=w137, "error in"=w139, "Main Test Status"=w141) -> ("queue out"=w144:refnum<queue>, "Main test sequence"=w142:T1, "output cluster"=w146:T4, "error out"=w143:errorcluster)  [unwired: 9 in]
      }
      frame "Emergancy Switch Check" {
        n41 = call "Result Comparison.vi"("input cluster"=w160) -> ("Output cluster"=w153:T4)  [unwired: 10 in, 4 out]
        n42 = call "Emergancy Switch .vi"() -> ("error out"=w152:errorcluster, "Command Response 2"=w151:string, "Result"=w149:string, "Pressed"=w150:bool)  [unwired: 8 in]
        n43 = call "Update_UI_Test_Sequence.vi"("queue out 2"=w148, "result"=w149, "input cluster"=w153, "Result"=w150, "measured value"=w151, "error in"=w152, "Main Test Status"=w154) -> ("queue out"=w157:refnum<queue>, "Main test sequence"=w155:T1, "output cluster"=w159:T4, "error out"=w156:errorcluster)  [unwired: 9 in]
      }
      frame "Update WIFI credentials " {
        n44 = call "WIFI_Cred.vi"() -> ("error out"=w165:errorcluster, "Command Response"=w164:string, "Result"=w162:string, "RESULT"=w163:bool)  [unwired: 8 in]
        n45 = call "Result Comparison.vi"("input cluster"=w173) -> ("Output cluster"=w166:T4)  [unwired: 10 in, 4 out]
        n46 = call "Update_UI_Test_Sequence.vi"("queue out 2"=w161, "result"=w162, "input cluster"=w166, "Result"=w163, "measured value"=w164, "error in"=w165, "Main Test Status"=w167) -> ("queue out"=w170:refnum<queue>, "Main test sequence"=w168:T1, "output cluster"=w172:T4, "error out"=w169:errorcluster)  [unwired: 9 in]
      }
      frame "Reboot" {
        n47 = disable-structure shown="Disabled" {
          disable-tunnel: [w190 _] -> w178
          disable-tunnel: [w189 _] -> w177
          disable-tunnel: [w188 _] -> w176
          disable-tunnel: [w187 _] -> w175
          frame Disabled {
            n48 = call "Reboot.vi"() -> ("error out"=w190:errorcluster, "Command Response"=w189:string, "Result"=w187:string, "RESULT"=w188:bool)  [unwired: 8 in]
          }
          frame Enabled {
          }
        }
        n49 = call "Result Comparison.vi"("input cluster"=w186) -> ("Output cluster"=w179:T4)  [unwired: 10 in, 4 out]
        n50 = call "Update_UI_Test_Sequence.vi"("queue out 2"=w174, "result"=w175, "input cluster"=w179, "Result"=w176, "measured value"=w177, "error in"=w178, "Main Test Status"=w180) -> ("queue out"=w183:refnum<queue>, "Main test sequence"=w181:T1, "output cluster"=w185:T4, "error out"=w182:errorcluster)  [unwired: 9 in]
      }
      frame "Unlock Opensesame & Stop_console Logs" {
        n51 = disable-structure shown="Disabled" {
          disable-tunnel: [w205 _] -> w194
          disable-tunnel: [w204 _] -> w193
          disable-tunnel: [w203 _] -> w192
          frame Disabled {
            n52 = call "Reboot Power Reset .vi"() -> ("error out"=w205:errorcluster, 2:"Result"=w204:string, 3:"Result"=w203:bool)  [unwired: 9 in]
          }
          frame Enabled {
          }
        }
        n53 = call "Result Comparison.vi"("input cluster"=w202) -> ("Output cluster"=w195:T4)  [unwired: 10 in, 4 out]
        n54 = call "Update_UI_Test_Sequence.vi"("queue out 2"=w191, "result"=w193, "input cluster"=w195, "Result"=w192, "error in"=w194, "Main Test Status"=w196) -> ("queue out"=w199:refnum<queue>, "Main test sequence"=w197:T1, "output cluster"=w201:T4, "error out"=w198:errorcluster)  [unwired: 10 in]
      }
      frame "WIFI State" {
        n55 = call "Result Comparison.vi"("input cluster"=w218) -> ("Output cluster"=w211:T4)  [unwired: 10 in, 4 out]
        n56 = call "WIFI_CON.vi"() -> ("error out"=w210:errorcluster, "Command Response"=w209:string, "Result"=w207:string, "RESULT"=w208:bool)  [unwired: 8 in]
        n57 = call "Update_UI_Test_Sequence.vi"("queue out 2"=w206, "result"=w207, "input cluster"=w211, "Result"=w208, "measured value"=w209, "error in"=w210, "Main Test Status"=w212) -> ("queue out"=w215:refnum<queue>, "Main test sequence"=w213:T1, "output cluster"=w217:T4, "error out"=w214:errorcluster)  [unwired: 9 in]
      }
      frame "WIFI SSID" {
        n58 = call "WIFI_SSID.vi"() -> ("error out"=w223:errorcluster, "Command Response"=w222:string, "Result"=w220:string, "RESULT"=w221:bool)  [unwired: 8 in]
        n59 = call "Result Comparison.vi"("input cluster"=w231) -> ("Output cluster"=w224:T4)  [unwired: 10 in, 4 out]
        n60 = call "Update_UI_Test_Sequence.vi"("queue out 2"=w219, "result"=w220, "input cluster"=w224, "Result"=w221, "measured value"=w222, "error in"=w223, "Main Test Status"=w225) -> ("queue out"=w228:refnum<queue>, "Main test sequence"=w226:T1, "output cluster"=w230:T4, "error out"=w227:errorcluster)  [unwired: 9 in]
      }
      frame "Board revision" {
        n61 = call "Result Comparison.vi"("input cluster"=w244) -> ("Output cluster"=w237:T4)  [unwired: 10 in, 4 out]
        n62 = call "Board version.vi"() -> ("error out"=w236:errorcluster, "Command Response"=w235:string, "Result"=w233:string, "RESULT"=w234:bool)  [unwired: 8 in]
        n63 = call "Update_UI_Test_Sequence.vi"("queue out 2"=w232, "result"=w233, "input cluster"=w237, "Result"=w234, "measured value"=w235, "error in"=w236, "Main Test Status"=w238) -> ("queue out"=w241:refnum<queue>, "Main test sequence"=w239:T1, "output cluster"=w243:T4, "error out"=w240:errorcluster)  [unwired: 9 in]
      }
      frame "ADC NTC Temp" {
        n64 = call "NTC Temp.vi"() -> ("error out"=w250:errorcluster, "Command Response"=w248:string, "number"=w251:dbl)  [unwired: 7 in, 2 out]
        n65 = call "Result Comparison.vi"("input cluster"=w259, "measured data"=w251, "error in (no error)"=w250) -> ("Output cluster"=w252:T4, "result"=w246:string, "result?"=w247:bool, "error out"=w249:errorcluster)  [unwired: 8 in, 1 out]
        n66 = call "Update_UI_Test_Sequence.vi"("queue out 2"=w245, "result"=w246, "input cluster"=w252, "Result"=w247, "measured value"=w248, "error in"=w249, "Main Test Status"=w253) -> ("queue out"=w256:refnum<queue>, "Main test sequence"=w254:T1, "output cluster"=w258:T4, "error out"=w255:errorcluster)  [unwired: 9 in]
      }
      frame "ADC_TYPE2_RCD_CURRENT" {
        n67 = call "ADT RCD Current.vi"() -> ("error out"=w265:errorcluster, "Command Response"=w264:string, "number"=w263:dbl)  [unwired: 7 in, 1 out]
        n68 = call "Result Comparison.vi"("input cluster"=w273, "measured data"=w263) -> ("Output cluster"=w266:T4, "result"=w262:string, "result?"=w261:bool)  [unwired: 9 in, 2 out]
        n69 = call "Update_UI_Test_Sequence.vi"("queue out 2"=w260, "result"=w262, "input cluster"=w266, "Result"=w261, "measured value"=w264, "error in"=w265, "Main Test Status"=w267) -> ("queue out"=w270:refnum<queue>, "Main test sequence"=w268:T1, "output cluster"=w272:T4, "error out"=w269:errorcluster)  [unwired: 9 in]
      }
      frame "5V Output Voltage" {
        n70 = call "Result Comparison.vi"("input cluster"=w285) -> ("Output cluster"=w276:T4, "measured value"=w282:string)  [unwired: 10 in, 3 out]
        n71 = call "Update_UI_Test_Sequence.vi"("queue out 2"=w274, "result"="PASS", "input cluster"=w276, "Result"=TRUE, "measured value"=w282, "Main Test Status"=w277) -> ("queue out"=w281:refnum<queue>, "Main test sequence"=w278:T1, "output cluster"=w284:T4, "error out"=w280:errorcluster)  [unwired: 10 in]
      }
      frame "3.3V Output Voltage" {
        n72 = call "Result Comparison.vi"("input cluster"=w296) -> ("Output cluster"=w289:T4)  [unwired: 10 in, 4 out]
        n73 = call "Update_UI_Test_Sequence.vi"("queue out 2"=w286, "input cluster"=w289, "Result"=TRUE, "measured value"="PASS", "Main Test Status"=w290) -> ("queue out"=w293:refnum<queue>, "Main test sequence"=w291:T1, "output cluster"=w295:T4, "error out"=w292:errorcluster)  [unwired: 11 in]
      }
      frame "D+M Sense" {
        n74 = disable-structure shown="Disabled" {
          frame Disabled {
            n75 = call "D+M Sense.vi"() -> ()  [unwired: 9 in, 3 out]
          }
          frame Enabled {
          }
        }
        n76 = call "Result Comparison.vi"("input cluster"=w307) -> ("Output cluster"=w300:T4)  [unwired: 10 in, 4 out]
        n77 = call "Update_UI_Test_Sequence.vi"("queue out 2"=w297, "input cluster"=w300, "Result"=TRUE, "measured value"="PASS", "Main Test Status"=w301) -> ("queue out"=w304:refnum<queue>, "Main test sequence"=w302:T1, "output cluster"=w306:T4, "error out"=w303:errorcluster)  [unwired: 11 in]
      }
      frame "Output Weld Sense" {
        n78 = call "Output Weld Detection.vi"() -> ("error out"=w315:errorcluster, "Command Response"=w313:string, "number"=w314:dbl, "Number"=w308:string)  [unwired: 5 in, 1 out]
        n79 = call "Result Comparison.vi"("input cluster"=w323, "measured data"=w314, "Measued String"=w308, "error in (no error)"=w315) -> ("Output cluster"=w316:T4, "result"=w310:string, "result?"=w311:bool, "error out"=w312:errorcluster)  [unwired: 7 in, 1 out]
        n80 = call "Update_UI_Test_Sequence.vi"("queue out 2"=w309, "result"=w310, "input cluster"=w316, "Result"=w311, "measured value"=w313, "error in"=w312, "Main Test Status"=w317) -> ("queue out"=w320:refnum<queue>, "Main test sequence"=w318:T1, "output cluster"=w322:T4, "error out"=w319:errorcluster)  [unwired: 9 in]
      }
      frame "FW Power Reset" {
        n81 = call "Result Comparison.vi"("input cluster"=w334) -> ("Output cluster"=w326:T4)  [unwired: 10 in, 4 out]
        n82 = call "Update_UI_Test_Sequence.vi"("queue out 2"=w324, "result"="PASS", "input cluster"=w326, "Result"=TRUE, "Main Test Status"=w327) -> ("queue out"=w331:refnum<queue>, "Main test sequence"=w328:T1, "output cluster"=w333:T4, "error out"=w330:errorcluster)  [unwired: 11 in]
      }
      frame "Unlock Opensesame & Stop console_Logs" {
        n83 = disable-structure shown="Disabled" {
          disable-tunnel: [w349 _] -> w338
          disable-tunnel: [w348 _] -> w337
          disable-tunnel: [w347 _] -> w336
          frame Disabled {
            n84 = call "Reboot Power Reset .vi"() -> ("error out"=w349:errorcluster, 2:"Result"=w348:string, 3:"Result"=w347:bool)  [unwired: 9 in]
          }
          frame Enabled {
          }
        }
        n85 = call "Result Comparison.vi"("input cluster"=w346) -> ("Output cluster"=w339:T4)  [unwired: 10 in, 4 out]
        n86 = call "Update_UI_Test_Sequence.vi"("queue out 2"=w335, "result"=w337, "input cluster"=w339, "Result"=w336, "error in"=w338, "Main Test Status"=w340) -> ("queue out"=w343:refnum<queue>, "Main test sequence"=w341:T1, "output cluster"=w345:T4, "error out"=w342:errorcluster)  [unwired: 10 in]
      }
      frame "Reset switch Check" {
        n87 = call "Reset Switch Power Reset .vi"() -> ("error out"=w353:errorcluster, 2:"Result"=w352:string, 3:"Result"=w351:bool)  [unwired: 9 in]
        n88 = call "Result Comparison.vi"("input cluster"=w361) -> ("Output cluster"=w354:T4)  [unwired: 10 in, 4 out]
        n89 = call "Update_UI_Test_Sequence.vi"("queue out 2"=w350, "result"=w352, "input cluster"=w354, "Result"=w351, "error in"=w353, "Main Test Status"=w355) -> ("queue out"=w358:refnum<queue>, "Main test sequence"=w356:T1, "output cluster"=w360:T4, "error out"=w357:errorcluster)  [unwired: 10 in]
      }
      frame "Exit" {
        (unwired) string[][] [] ("Test status item names")
        n90 = disable-structure shown="Enabled" {
          disable-tunnel: w367 -> [w372 w375]
          disable-tunnel: [w371 w375] -> w364
          frame Disabled {
            n91 = call "Result Comparison.vi"("input cluster"=w372, "Measued String"="0") -> ("Output cluster"=w374:T4, "result"=w370:string, "measured value"=w369:string, "result?"=w373:bool)  [unwired: 9 in, 1 out]
            n92 = call "Update_UI_Test_Sequence.vi"("Result"=w373, "measured value"=w369, "result"=w370, "input cluster"=w374) -> ("output cluster"=w371:T7)  [unwired: 2 in, 5 out]
          }
          frame Enabled {
          }
        }
        n93 = Unbundle By Name(w364) -> ("UI"=→"Result":string[][])
      }
    }
    n94 = call "Update Listbox Row.vi"("cluster in"=w19) -> ("cluster out"=w20:T4)  [unwired: 10 in]
  }
  n95 = Release Queue(queue=w8, error in (no error)=w7) -> (error out=w9:errorcluster)  [unwired: 1 in, 2 out]
  n96 = call <vilib>:"Clear Errors.vi"("error in (no error)"=w9) -> ()  [unwired: 5 in, 2 out]
